vi "zadanie_2_lab0.vi"() -> ()   [LabVIEW 2020]
uses:
  <vilib>/numeric/Random Number (Range) U64.vi
  <vilib>/numeric/sub_Random U32.vi
panel:
  out "Waveform Graph":u64[](graph)
  out "Waveform Chart":u64[](graph)
  out "wylosowany numer":u64
  in  "Zatrzymaj losowanie":bool
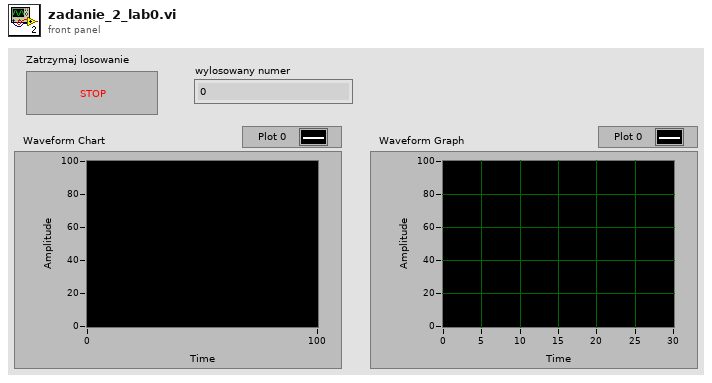
[diagram p1: front panel]
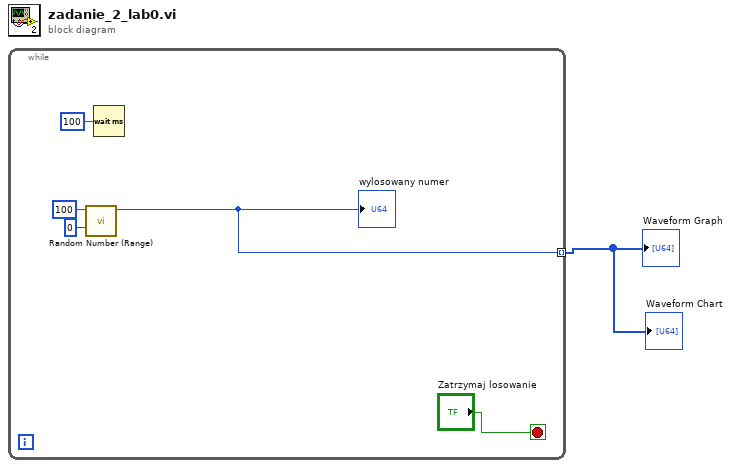
[diagram p0: block diagram]
diagram:
  n1 = while {
    tunnel: [w2] -> w1 mode=indexing
    stop <- "Zatrzymaj losowanie" stop-if-true
    n2 = call-poly <vilib>:"Random Number (Range).vi"("lower bound (0)"=u64 0, "upper bound (100)"=u64 100) -> ("number"=w2:u64)  [unwired: 9 in]
    "wylosowany numer" <- w2
    n3 = Wait (ms)(milliseconds to wait=u32 100) -> ()  [unwired: 1 out]
  }
  "Waveform Graph" <- w1
  "Waveform Chart" <- w1
